vi "Laser.vi"(8 "error in (no error)":errorcluster, 10 "Temp (C)":dbl, 11 "Current (A)":dbl) -> (0 "error out":errorcluster, 2 "Ith (A)":dbl, 3 "Power (W)":dbl)   [LabVIEW 2026]
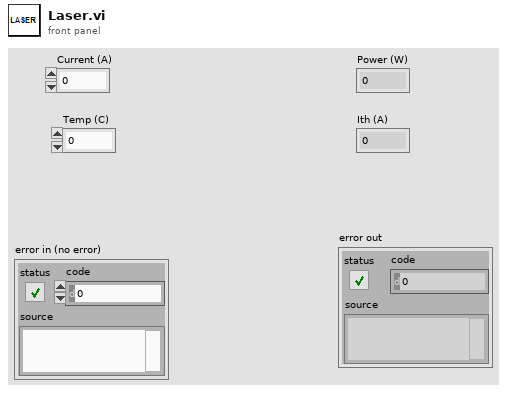
[diagram p1: front panel]
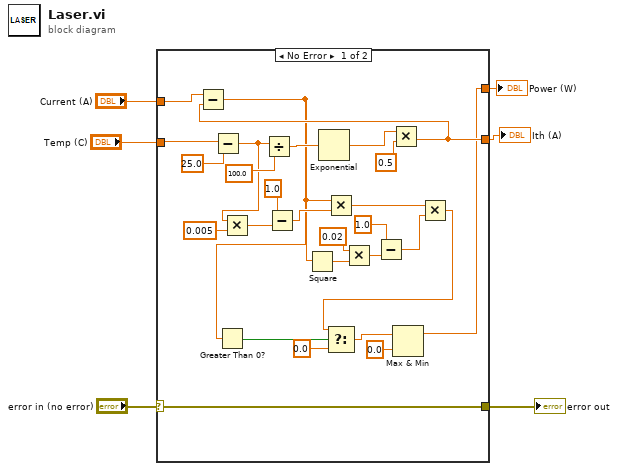
[diagram p0: block diagram]
diagram:
  n1 = case shown="No Error" "error in (no error)" {
    selector: "error in (no error)" -> [w7 w34]
    tunnel: [w22 _] -> w4
    tunnel: "Temp (C)" -> [w28 _]
    tunnel: "Current (A)" -> [w23 _]
    tunnel: [w8 _] -> w2
    tunnel: [w7 w34] -> w1
    frame No Error {
      n2 = Subtract(x=w28, y=25.0) -> (x-y=w26:dbl)
      n3 = Multiply(x=w26, y=0.005 ("x-y")) -> (x*y=w25:dbl)
      n4 = Divide(x=w26, y=100.0) -> (x/y=w31:dbl)
      n5 = Subtract(x=1.0, y=w25) -> (x-y=w21:dbl)
      n6 = Exponential(1:w31) -> (0:w30:dbl)
      n7 = Multiply(x=w30, y=0.5) -> (x*y=w22:dbl)
      n8 = Subtract(x=w23, y=w22) -> (x-y=w14:dbl)
      n9 = Greater Than 0?(x=w14) -> (x > 0?=w13:bool)
      n10 = Square(x=w14) -> (x^2=w20:dbl)
      n11 = Multiply(x=w14, y=w21) -> (x*y=w16:dbl)
      n12 = Multiply(x=0.02, y=w20) -> (x*y=w18:dbl)
      n13 = Subtract(x=1.0, y=w18) -> (x-y=w15:dbl)
      n14 = Multiply(x=w16, y=w15) -> (x*y=w12:dbl)
      n15 = Select(t=w12, s=w13, f=0.0) -> (s? t:f=w10:dbl)
      n16 = Max & Min(x=w10, y=0.0) -> (max(x,y)=w8:dbl)  [unwired: 1 out]
    }
    frame Error {
    }
  }
  "Power (W)" <- w2
  "Ith (A)" <- w4
  "error out" <- w1
